vi "HostMem Clone.vi"(8 "error in (no error)":errorcluster, 11 "HostMem in":refnum<class "HostMem.lvclass">) -> (0 "error out":errorcluster, 2 "Clone out":refnum<class "HostMem.lvclass">, 3 "HostMem out":refnum<class "HostMem.lvclass">)   [LabVIEW 2020, in "OpenLvVision_OpenCv.lvlib" / "Cuda.lvlib" / "HostMem.lvclass"]
doc: "Returns deep copy of the matrix, i.e. the data is copied"
uses:
  HostMem.lvclass
  C:/Users/lukas/Documents/OpenLvVision_OpenCv/SourceCode/LabView/OpenLvVision_OpenCv/_LvHelpers/EdvrObject/EdvrObject.lvclass
  _LvHelpers/EdvrObject/EdvrObject.lvclass/EdvrObject.ctl
  _LvHelpers/EdvrObject/TypeDef/Edvr.ctl
  OpenLvVision_OpenCv.lvlib
  <vilib>/Utility/error.llb/Error Cluster From Error Code.vi
  <vilib>/ErrorRing/Error Ring.xnode
  _LvHelpers/EdvrObject/EdvrObject.lvclass
  Dlls/OlvOpenCvWrapper.dll
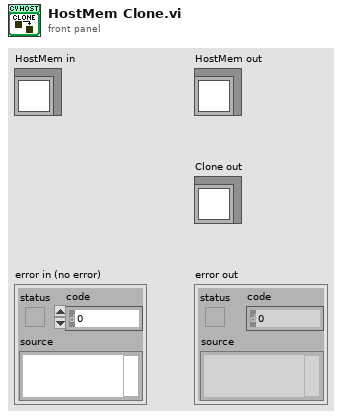
[diagram p1: front panel]
types:
  T1 = typedef "OpenLvVision_OpenCv.lvlib/EdvrObject.lvclass/Edvr.ctl" = refnum<data-value>
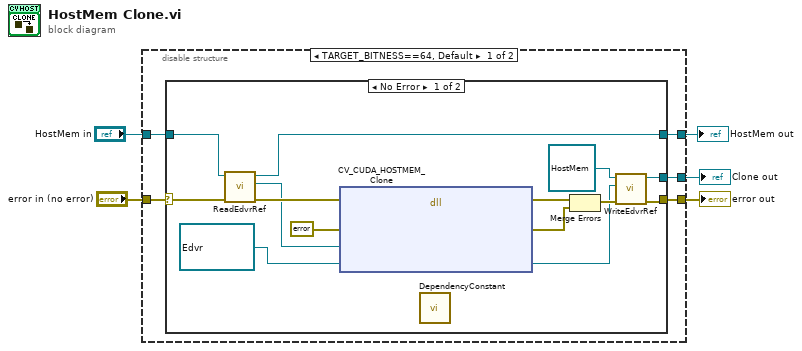
[diagram p0: block diagram]
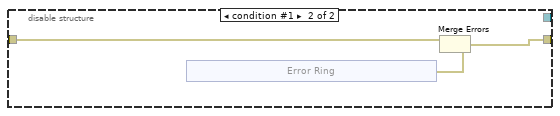
[diagram p3: hidden frame]
diagram:
  n1 = disable-structure shown="TARGET_BITNESS==64, Default" {
    disable-tunnel: "error in (no error)" -> [w10 w28]
    disable-tunnel: [w9 w29] -> w4
    disable-tunnel: "HostMem in" -> [w8 _]
    disable-tunnel: [w7 _] -> w2
    disable-tunnel: [w6 _] -> w1
    frame condition #0 (active) {
      n2 = case shown="No Error" w10 {
        selector: w10 -> [w17 w26]
        tunnel: [w14 w26] -> w9
        tunnel: w8 -> [w21 w25]
        tunnel: [w18 w25] -> w7
        tunnel: [w11 _] -> w6
        frame No Error {
          n3 = call "ReadEdvrRef.vi"("error in (no error)"=w17, "EdvrObject in"=w21) -> ("error out"=w20:errorcluster, "Edvr"=w19:T1, "EdvrObject out"=w18:refnum<class "HostMem.lvclass">)  [unwired: 7 in]
          n4 = dll-call lib="C:/Users/lukas/Documents/OpenLvVision_OpenCv/SourceCode/LabView/OpenLvVision_OpenCv/Dlls/OlvOpenCvWrapper.dll" fn="CV_CUDA_HOSTMEM_Clone"(error in=w20, "Error"=errorcluster {"status"=FALSE, "code"=0, "source"=""} ("error out"), "edvrRefSrc"=w19, "edvrRefDst"=T1 refnum ("Edvr")) -> (error out=w24:errorcluster, "Error"=w23:errorcluster, "edvrRefDst"=w12:T1)  [unwired: 4 in, 1 out]
          n5 = call "DependencyConstant.vi"() -> ()  [unwired: 12 in]
          n6 = Merge Errors(w24, w23) -> (w15:errorcluster)
          n7 = call "WriteEdvrRef.vi"("error in (no error)"=w15, "Edvr"=w12, "EdvrObject in"=refnum<class "HostMem.lvclass"> refnum ("Dst out")) -> ("error out"=w14:errorcluster, "EdvrObject out"=w11:refnum<class "HostMem.lvclass">)  [unwired: 7 in]
        }
        frame Error {
        }
      }
    }
    frame condition #1 {
      n8 = xnode "Error Ring"() -> ("error out"=w27:errorcluster)
      n9 = Merge Errors(w28, w27) -> (w29:errorcluster)
    }
  }
  "error out" <- w4
  "HostMem out" <- w2
  "Clone out" <- w1
